vi "Update graph data.vi"(8 "error in (no error)":errorcluster, 10 "Acquisition data":T2, 11 "Graph data":T1) -> (0 "error out":errorcluster, 3 "Graph data":T1)   [LabVIEW 2020]
uses:
  controls/Acquisition data --typedef.ctl
  controls/Graph data --typedef.ctl
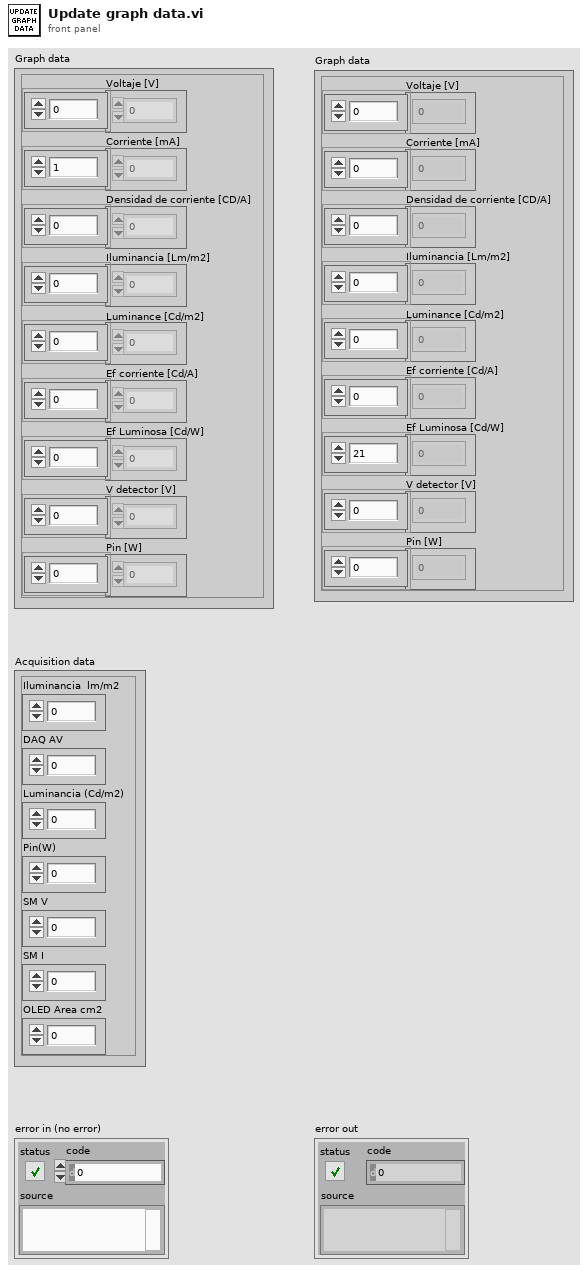
[diagram p1: front panel]
types:
  T1 = typedef "Graph data --typedef.ctl" = cluster{"Voltaje [V]":dbl[], "Corriente [mA]":dbl[], "Densidad de corriente [CD/A]":dbl[], "Iluminancia [Lm/m2]":dbl[], "Luminance [Cd/m2]":dbl[], "Ef corriente [Cd/A]":dbl[], "Ef Luminosa [Cd/W]":dbl[], "V detector [V]":dbl[], "Pin [W]":dbl[]}
  T2 = typedef "Acquisition data --typedef.ctl" = cluster{"Iluminancia  lm/m2":dbl, "DAQ AV":dbl, "Luminancia (Cd/m2)":dbl, "Pin(W)":dbl, "SM V":dbl, "SM I":dbl, "OLED Area cm2":dbl}
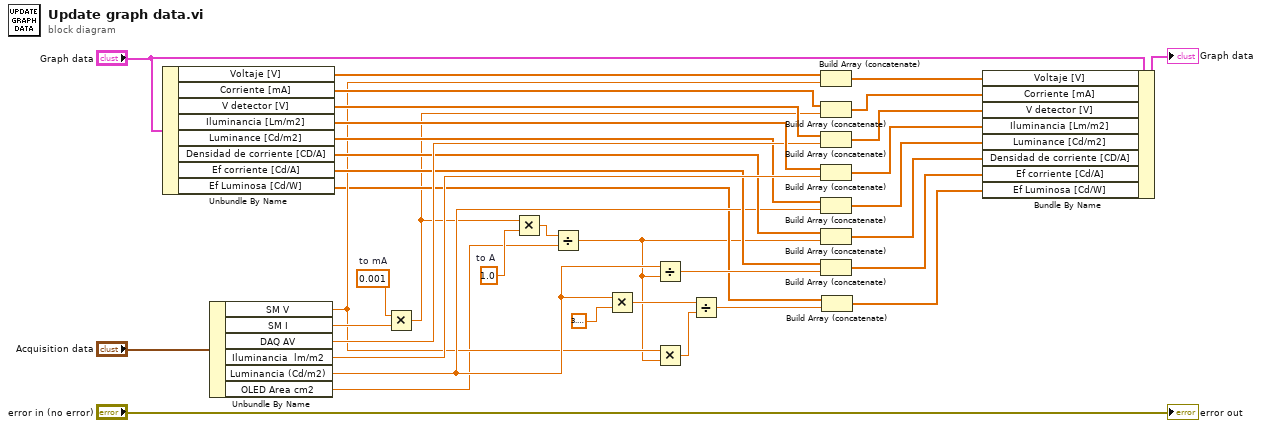
[diagram p0: block diagram]
diagram:
  w2 = 1.0  # to A
  w5 = 0.001  # to mA
  n1 = Unbundle By Name("Graph data") -> ("Voltaje [V]"=w32:dbl[], "Corriente [mA]"=w30:dbl[], "V detector [V]"=w29:dbl[], "Iluminancia [Lm/m2]"=w28:dbl[], "Luminance [Cd/m2]"=w22:dbl[], "Densidad de corriente [CD/A]"=w20:dbl[], "Ef corriente [Cd/A]"=w17:dbl[], "Ef Luminosa [Cd/W]"=w8:dbl[])
  n2 = Unbundle By Name("Acquisition data") -> ("SM V"=w11:dbl, "SM I"=w19:dbl, "DAQ AV"=w27:dbl, "Iluminancia  lm/m2"=w23:dbl, "Luminancia (Cd/m2)"=w13:dbl, "OLED Area cm2"=w1:dbl)
  n3 = Multiply(x=w5, y=w19) -> (x*y=w6:dbl)
  n4 = Multiply(x=w6, y=w2) -> (x*y=w3:dbl)
  n5 = Divide(x=w3, y=w1) -> (x/y=w4:dbl)
  n6 = Multiply(x=w13, y=3.141592653589793) -> (x*y=w12:dbl)
  n7 = Divide(x=w13, y=w4) -> (x/y=w16:dbl)
  n8 = Multiply(x=w11, y=w4) -> (x*y=w10:dbl)
  n9 = Divide(x=w12, y=w10) -> (x/y=w9:dbl)
  n10 = Build Array (concatenate)(w32, w11) -> (w31:dbl[])
  n11 = Build Array (concatenate)(w30, w6) -> (w26:dbl[])
  n12 = Build Array (concatenate)(w29, w27) -> (w25:dbl[])
  n13 = Build Array (concatenate)(w28, w23) -> (w24:dbl[])
  n14 = Build Array (concatenate)(w22, w13) -> (w21:dbl[])
  n15 = Build Array (concatenate)(w20, w4) -> (w18:dbl[])
  n16 = Build Array (concatenate)(w17, w16) -> (w15:dbl[])
  n17 = Build Array (concatenate)(w8, w9) -> (w7:dbl[])
  n18 = Bundle By Name(cluster="Graph data", "Voltaje [V]"=w31, "Corriente [mA]"=w26, "V detector [V]"=w25, "Iluminancia [Lm/m2]"=w24, "Luminance [Cd/m2]"=w21, "Densidad de corriente [CD/A]"=w18, "Ef corriente [Cd/A]"=w15, "Ef Luminosa [Cd/W]"=w7) -> (→"Graph data":T1)
  "error out" <- "error in (no error)"
